vi "Output Parameter Cluster Label--constant.vi"() -> (3 "Output Parameter Cluster Label":string)   [LabVIEW 2026]
doc: "This constant defines the label of output parameter control (as a format string)."
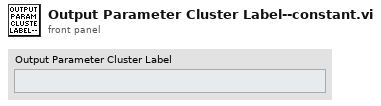
[diagram p1: front panel]
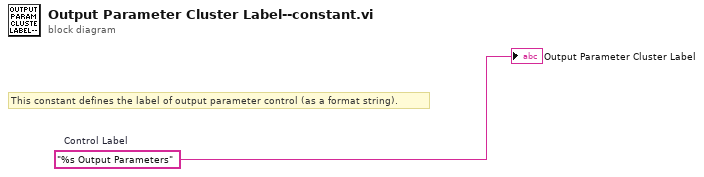
[diagram p0: block diagram]
diagram:
  w1 = "%s Output Parameters"  # Control Label
  # "This constant defines the label of output parameter control (as a format string)."
  "Output Parameter Cluster Label" <- w1
